vi "ReadWave.vi"() -> ()   [LabVIEW 2015]
panel:
  in  "组合框":string(combo)="电压数据"
  out "波形图":dbl[](graph)
  out "数组":dbl[](array[numeric])
  out "读取缓冲区":string
  in  "读取的字节数":u32=102400
  in  "VISA资源名称":refnum<visa-resource-name>
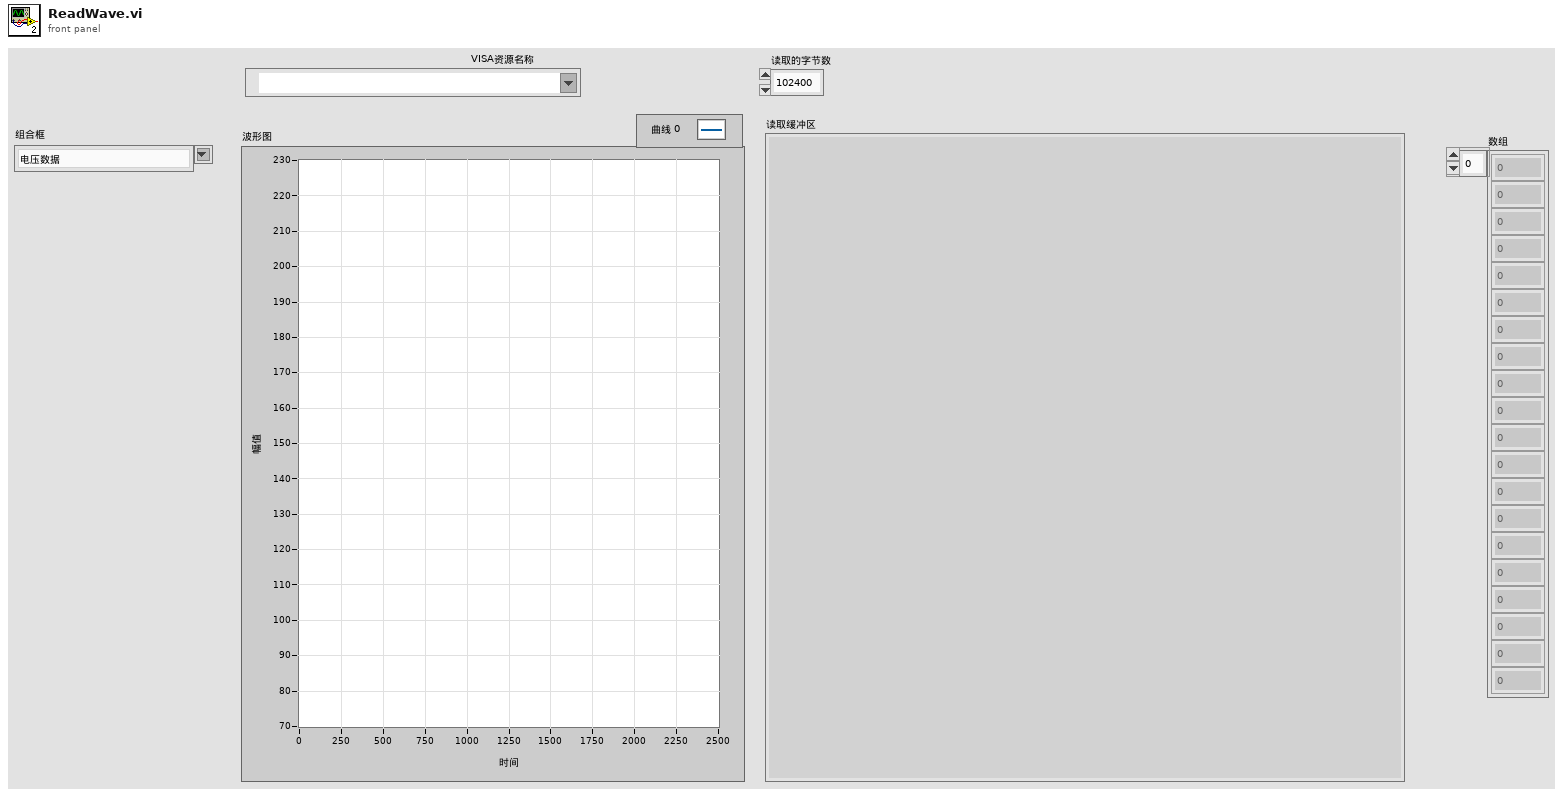
[diagram p1: front panel]
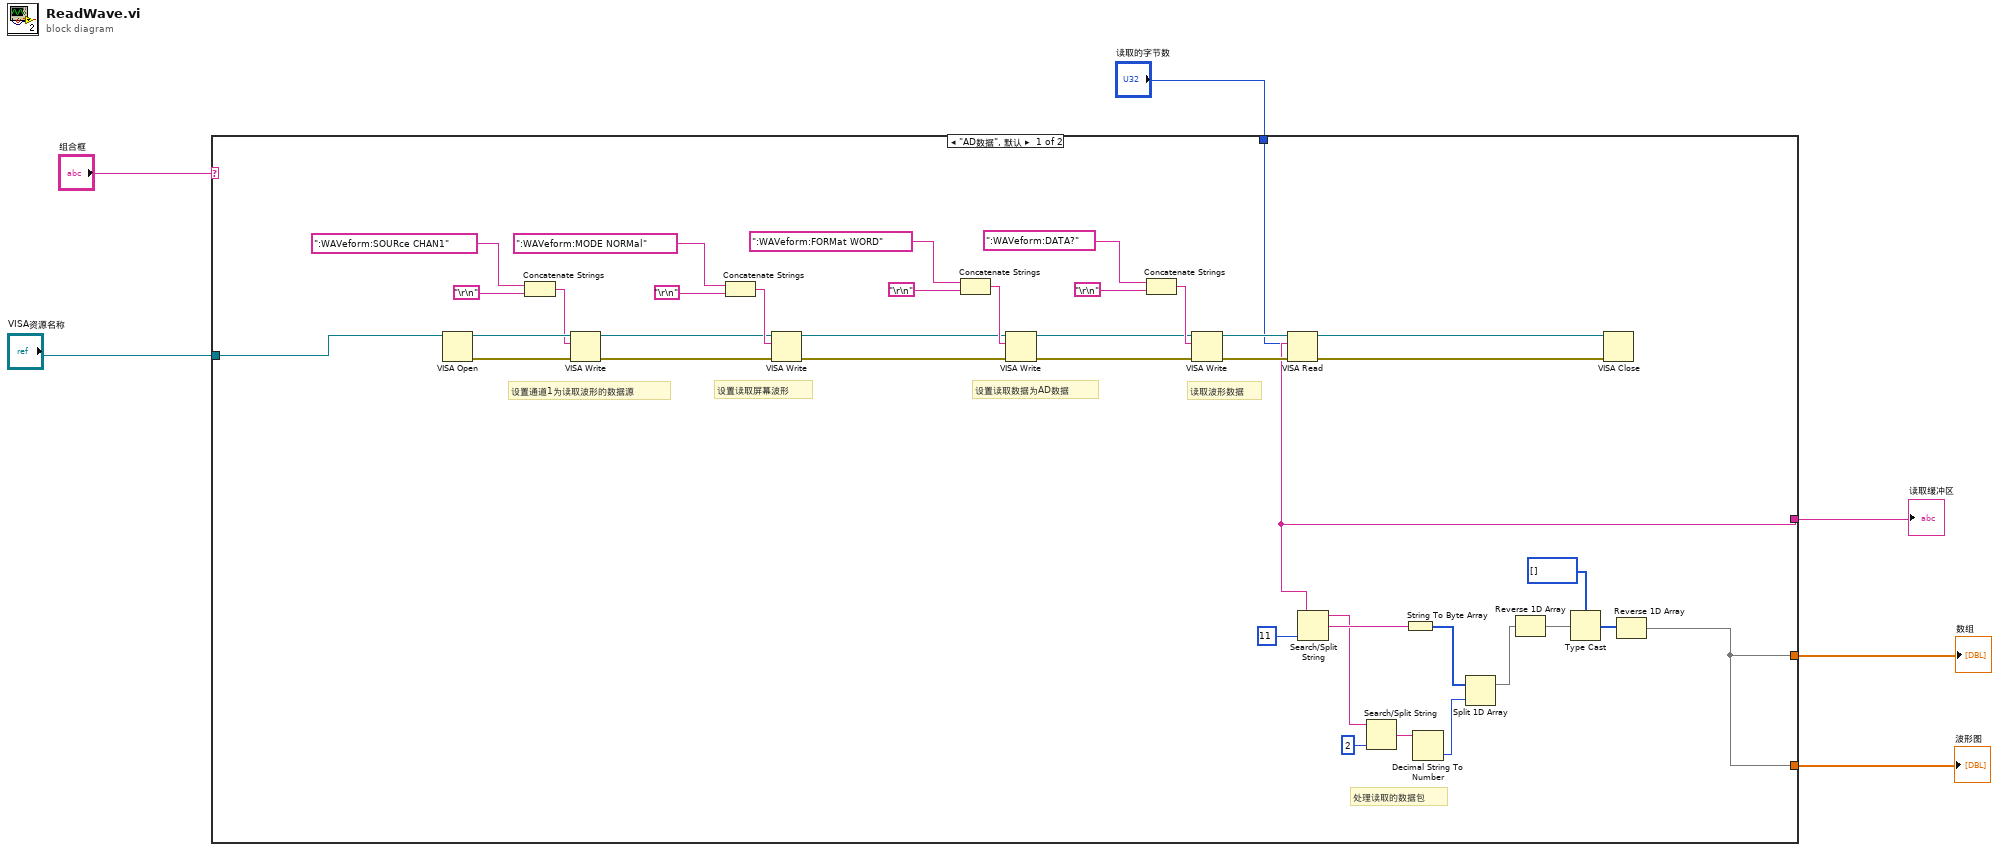
[diagram p0: block diagram]
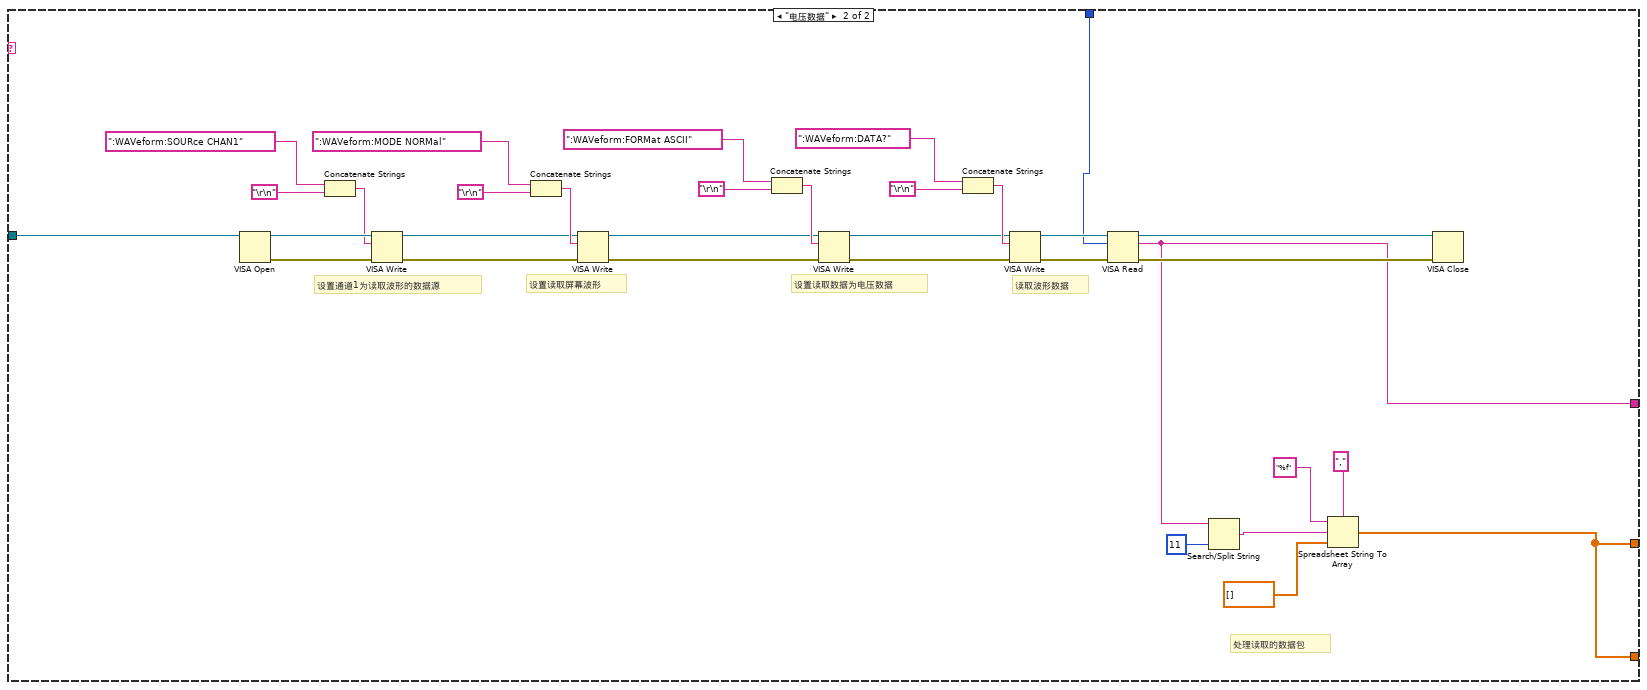
[diagram p2: hidden frame]
diagram:
  n1 = case shown="\"AD数据\", 默认" "组合框" {
    tunnel: [w7 w49] -> w5
    tunnel: [w7 w49] -> w4
    tunnel: [w20 w48] -> w3
    tunnel: "VISA资源名称" -> [w19 w47]
    tunnel: "读取的字节数" -> [w18 w46]
    frame "AD数据", Default {
      # "处理读取的数据包"
      # "读取波形数据"
      # "设置读取数据为AD数据"
      # "设置读取屏幕波形"
      # "设置通道1为读取波形的数据源"
      n2 = VISA Open(VISA resource name=w19) -> (VISA resource name=w45:refnum<visa-resource-name>, error out=w41:errorcluster)  [unwired: 4 in]
      n3 = Concatenate Strings(":WAVeform:SOURce CHAN1" ("字符串"), "\r\n") -> (w42:string)
      n4 = VISA Write(VISA resource name=w45, write buffer=w42, error in (no error)=w41) -> (VISA resource name out=w35:refnum<visa-resource-name>, error out=w34:errorcluster)  [unwired: 1 out]
      n5 = Concatenate Strings(":WAVeform:MODE NORMal" ("字符串"), "\r\n") -> (w37:string)
      n6 = VISA Write(VISA resource name=w35, write buffer=w37, error in (no error)=w34) -> (VISA resource name out=w30:refnum<visa-resource-name>, error out=w29:errorcluster)  [unwired: 1 out]
      n7 = Concatenate Strings(":WAVeform:FORMat WORD" ("字符串"), "\r\n") -> (w32:string)
      n8 = VISA Write(VISA resource name=w30, write buffer=w32, error in (no error)=w29) -> (VISA resource name out=w25:refnum<visa-resource-name>, error out=w24:errorcluster)  [unwired: 1 out]
      n9 = Concatenate Strings(":WAVeform:DATA?" ("字符串"), "\r\n") -> (w27:string)
      n10 = VISA Write(VISA resource name=w25, write buffer=w27, error in (no error)=w24) -> (VISA resource name out=w23:refnum<visa-resource-name>, error out=w22:errorcluster)  [unwired: 1 out]
      n11 = VISA Read(VISA resource name=w23, byte count=w18, error in (no error)=w22) -> (VISA resource name out=w44:refnum<visa-resource-name>, read buffer=w20:string, error out=w40:errorcluster)  [unwired: 1 out]
      n12 = Search/Split String(string=w20, offset (0)=11 ("偏移量(0)")) -> (substring before match=w14:string, match + rest of string=w17:string)  [unwired: 1 in, 1 out]
      n13 = Search/Split String(string=w14, offset (0)=2 ("偏移量(0)")) -> (match + rest of string=w12:string)  [unwired: 1 in, 2 out]
      n14 = String To Byte Array(string=w17) -> (unsigned byte array=w11:u8[])
      n15 = Decimal String To Number(string=w12) -> (number=w10:i32)  [unwired: 2 in, 1 out]
      n16 = Split 1D Array(array=w11, index=w10) -> (first subarray=w9:u8[])  [unwired: 1 out]
      n17 = Reverse 1D Array(array=w9) -> (reversed array=w15:u8[])
      n18 = Type Cast(type=u16[] [], x=w15) -> (*(type *) &x=w8:u16[])
      n19 = VISA Close(VISA resource name=w44, error in (no error)=w40) -> ()  [unwired: 1 out]
      n20 = Reverse 1D Array(array=w8) -> (reversed array=w7:u16[])
    }
    frame "电压数据" {
      # "处理读取的数据包"
      # "读取波形数据"
      # "设置读取数据为电压数据"
      # "设置读取屏幕波形"
      # "设置通道1为读取波形的数据源"
      n21 = VISA Open(VISA resource name=w47) -> (VISA resource name=w78:refnum<visa-resource-name>, error out=w74:errorcluster)  [unwired: 4 in]
      n22 = Concatenate Strings(":WAVeform:SOURce CHAN1" ("字符串"), "\r\n") -> (w75:string)
      n23 = VISA Write(VISA resource name=w78, write buffer=w75, error in (no error)=w74) -> (VISA resource name out=w68:refnum<visa-resource-name>, error out=w67:errorcluster)  [unwired: 1 out]
      n24 = Concatenate Strings(":WAVeform:MODE NORMal" ("字符串"), "\r\n") -> (w70:string)
      n25 = VISA Write(VISA resource name=w68, write buffer=w70, error in (no error)=w67) -> (VISA resource name out=w63:refnum<visa-resource-name>, error out=w62:errorcluster)  [unwired: 1 out]
      n26 = Concatenate Strings(":WAVeform:FORMat ASCII" ("字符串"), "\r\n") -> (w65:string)
      n27 = VISA Write(VISA resource name=w63, write buffer=w65, error in (no error)=w62) -> (VISA resource name out=w58:refnum<visa-resource-name>, error out=w57:errorcluster)  [unwired: 1 out]
      n28 = Concatenate Strings(":WAVeform:DATA?" ("字符串"), "\r\n") -> (w60:string)
      n29 = VISA Write(VISA resource name=w58, write buffer=w60, error in (no error)=w57) -> (VISA resource name out=w56:refnum<visa-resource-name>, error out=w55:errorcluster)  [unwired: 1 out]
      n30 = VISA Read(VISA resource name=w56, byte count=w46, error in (no error)=w55) -> (VISA resource name out=w77:refnum<visa-resource-name>, read buffer=w48:string, error out=w73:errorcluster)  [unwired: 1 out]
      n31 = Search/Split String(string=w48, offset (0)=11 ("偏移量(0)")) -> (match + rest of string=w52:string)  [unwired: 1 in, 2 out]
      n32 = Spreadsheet String To Array(delimiter (Tab)="," ("分隔符(Tab)"), format string="%f" ("格式字符串"), spreadsheet string=w52, array type (2D Dbl)=dbl[] []) -> (array=w49:dbl[])
      n33 = VISA Close(VISA resource name=w77, error in (no error)=w73) -> ()  [unwired: 1 out]
    }
  }
  "数组" <- w4
  "波形图" <- w5
  "读取缓冲区" <- w3
